vi "Initialize SLSC Switch Engine.vi"(8 "error in (no error)":errorcluster, 11 "Device Ref in":T2 format="%.0x") -> (0 "error out":errorcluster, 1 "SLSC Switch Consumer out":refnum<class "SLSC Switch Consumer.lvclass">, 2 "FIFO Indices":T1, 3 "Device Ref out":T2 format="%.0x")   [LabVIEW 2020, in "SLSC Switch Engine.lvlib"]
uses:
  SLSC Switch Engine.lvlib
  <vilib>/NI VeriStand/Custom Device API/Custom Device Item Ref.ctl
  Includes/SLSCSwitchMessaging.lvlibp/SLSC Switch Consumer/SLSC Switch Consumer.lvclass
  Shared/FIFO Indices.ctl
  Shared/Compiled.Settings.ctl
  Shared/Communication Configuration.ctl
  Shared/Driver Configuration.ctl
  Includes/SLSCSwitchMessaging.lvlibp/SLSC Switch Init Parameters/SLSC Switch Init Parameters.lvclass
  C:/Users/nitest/Desktop/Git 2020/niveristand-routing-and-faulting-custom-device/Includes/CDMessaging.lvlibp/Parameters/Abstract Init Parameters/Abstract Init Parameters.lvclass
  C:/Users/nitest/Desktop/Git 2020/niveristand-routing-and-faulting-custom-device/Includes/CDMessaging.lvlibp/Switch/Abstract Switch Init Parameters/Abstract Switch Init Parameters.lvclass
  Includes/CDMessaging.lvlibp/Message Queue/Message Queue/Message Queue.lvclass
  C:/Users/nitest/Desktop/Git 2020/niveristand-routing-and-faulting-custom-device/Includes/CDMessaging.lvlibp/Message Queue/Abstract Message Queue/Abstract Message Queue.lvclass
  Shared/Constants.vi
  <vilib>/NI VeriStand/Custom Device API/Get Item Property (Variant).vi
  <vilib>/NI VeriStand/Custom Device API/Custom Device API.lvlib
  Shared/SLSC Switch Shared.lvlib
  Includes/CDMessaging.lvlibp/Consumer/Abstract Consumer/Abstract Consumer.lvclass
  C:/Users/nitest/Desktop/Git 2020/niveristand-routing-and-faulting-custom-device/Includes/CDMessaging.lvlibp/Consumer/Abstract Consumer/Abstract Consumer.lvclass
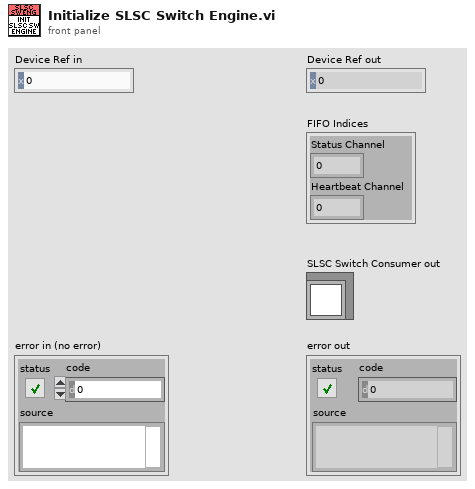
[diagram p1: front panel]
types:
  T1 = typedef "SLSC Switch Shared.lvlib/FIFO Indices.ctl" = cluster{"Status Channel":i32, "Heartbeat Channel":i32}
  T2 = typedef "Custom Device API.lvlib/Custom Device Item Ref.ctl" = u64
  T3 = typedef "SLSC Switch Shared.lvlib/Compiled.Settings.ctl" = cluster{"Custom Device Name":string, "Communication Configuration":T4, "Driver Configuration":T5, "FIFO Indices":T1}
  T4 = typedef "SLSC Switch Shared.lvlib/Communication Configuration.ctl" = cluster{"Consumer Queue Name":string}
  T5 = typedef "SLSC Switch Shared.lvlib/Driver Configuration.ctl" = cluster{"Topology":string, "Switches JSON":string, "Source Channels":string[], "Configuration Channels":string[], "Reservation Group":string}
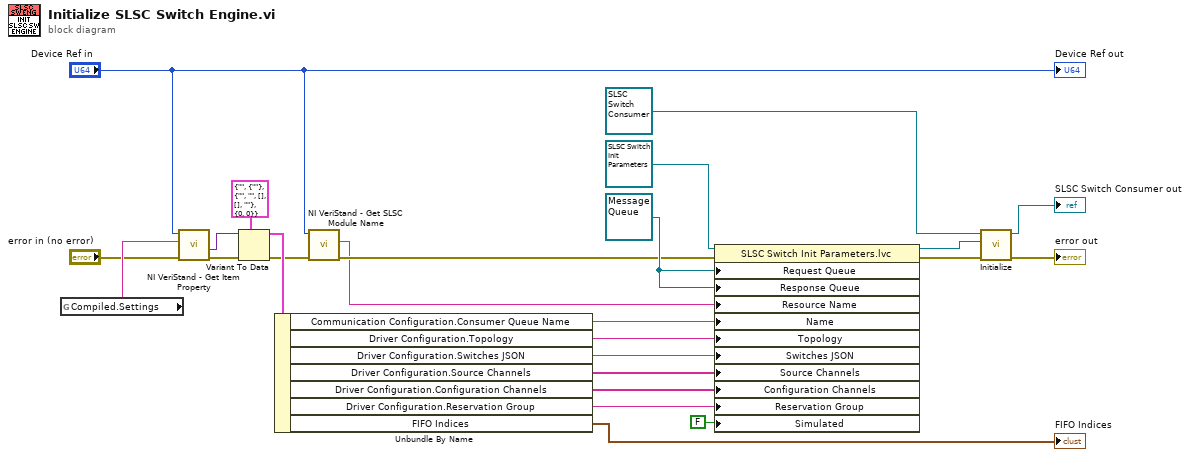
[diagram p0: block diagram]
diagram:
  w20 = refnum<class "Message Queue.lvclass"> refnum ("Request Queue")
  n1 = global read "Constants.vi" "Compiled.Settings"() -> (w25:string)
  n2 = call-poly <vilib>:"NI VeriStand - Get Item Property.vi"("error in (no error)"="error in (no error)", "Property Name"=w25, "Item Ref in"="Device Ref in") -> ("error out"=w24:errorcluster, "Value"=w23:variant)  [unwired: 5 in, 2 out]
  n3 = Variant To Data(error in=w24, type=T3 {"Custom Device Name"="", "Communication Configuration"={"Consumer Queue Name"=""}, "Driver Configuration"={"Topology"="", "Switches JSON"="", "Source Channels"=[], "Configuration Channels"=[], "Reservation Group"=""}, "FIFO Indices"={"Status Channel"=0, "Heartbeat Channel"=0}} ("Compiled.Settings"), Variant=w23) -> (data=w18:T3, error out=w6:errorcluster)
  n4 = Unbundle By Name(w18) -> ("Communication Configuration.Consumer Queue Name"=w3:string, "Driver Configuration.Topology"=w17:string, "Driver Configuration.Switches JSON"=w16:string, "Driver Configuration.Source Channels"=w8:string[], "Driver Configuration.Configuration Channels"=w7:string[], "Driver Configuration.Reservation Group"=w1:string, "FIFO Indices"=→"FIFO Indices":T1)
  n5 = call <vilib>:"NI VeriStand - Get SLSC Module Name.vi"("error in (no error)"=w6, "Item Ref in"="Device Ref in") -> ("error out"=w4:errorcluster, "SLSC Module"=w2:string)  [unwired: 7 in, 1 out]
  n6 = property class="SLSC Switch Init Parameters.lvc"(reference=refnum<class "SLSC Switch Init Parameters.lvclass"> refnum ("SLSC Switch Init Parameters"), error in=w4, "Request Queue"=w20, "Response Queue"=w20, "Resource Name"=w2, "Name"=w3, "Topology"=w17, "Switches JSON"=w16, "Source Channels"=w8, "Configuration Channels"=w7, "Reservation Group"=w1, "Simulated"=FALSE) -> (reference out=w13:refnum<class "SLSC Switch Init Parameters.lvclass">, error out=w15:errorcluster)
  n7 = call "Initialize.vi"("error in (no error)"=w15, "Parameters in"=w13, "Abstract Consumer in"=refnum<class "SLSC Switch Consumer.lvclass"> refnum ("SLSC Switch Consumer")) -> ("error out"=→"error out":errorcluster, "Abstract Consumer out"=→"SLSC Switch Consumer out":refnum<class "SLSC Switch Consumer.lvclass">)  [unwired: 7 in]
  "Device Ref out" <- "Device Ref in"
